vi "test elicitation.vi"(8 "error in (no error)":errorcluster) -> (0 "error out":errorcluster, 3 "body":string)   [LabVIEW 2020, in "MCP Server tests.lvlib"]
doc: "Elicitation with the multi round-trip pattern of MCP 2026-07-28. fake_tool_confirm calls Confirm With User.vi with the key confirm_action. A modern call from a client with the elicitation capability gets resultType input_required with inputRequests.confirm_action (elicitation/create, form mode); the retry with inputResponses accept runs the confirmed path, decline the declined path. Without the capability, and in the legacy era, the tool takes its not supported path. The requests are sent with the LabVIEW HTTP Client directly."
uses:
  MCP Server tests.lvlib
  <vilib>/JDP Science/JSONtext/Next JSON Value.vi
  <vilib>/JDP Science/JSONtext/String Subset.vi
  <vilib>/JDP Science/JSONtext/Parsing/Advance past next JSON Value (inlined COPY).vi
  <vilib>/JDP Science/JSONtext/Parsing/Advance past whitespace.vi
  <vilib>/JDP Science/JSONtext/Parsing/Advance past String.vi
  <vilib>/JDP Science/JSONtext/Parsing/Advance past Number.vi
  <vilib>/JDP Science/JSONtext/Parsing/Advance past Line Ending.vi
  <vilib>/JDP Science/JSONtext/Parsing/Parse Full Path or Item Name.vi
  <vilib>/JDP Science/JSONtext/Parsing/Advance past Array.vi
  <vilib>/JDP Science/JSONtext/Parsing/Advance past Object.vi
  <vilib>/JDP Science/JSONtext/support/Error Cluster From Code.vi
  <vilib>/JDP Science/JSONtext/Offset/Find Item Locations by Path.vi
  <vilib>/addons/_JKI Toolkits/Caraya/classes/Test/Test.lvclass
  <vilib>/JDP Science/JSONtext/JSONtext.lvlib
  <vilib>/addons/_JKI Toolkits/Caraya/classes/Assert/Assert.lvclass
panel:
  out "lookup error":errorcluster
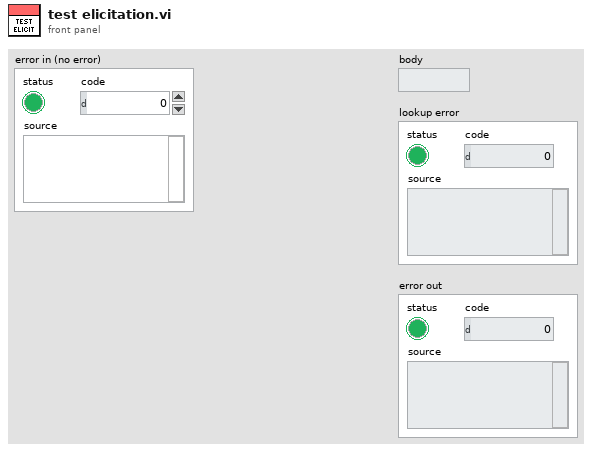
[diagram p1: front panel]
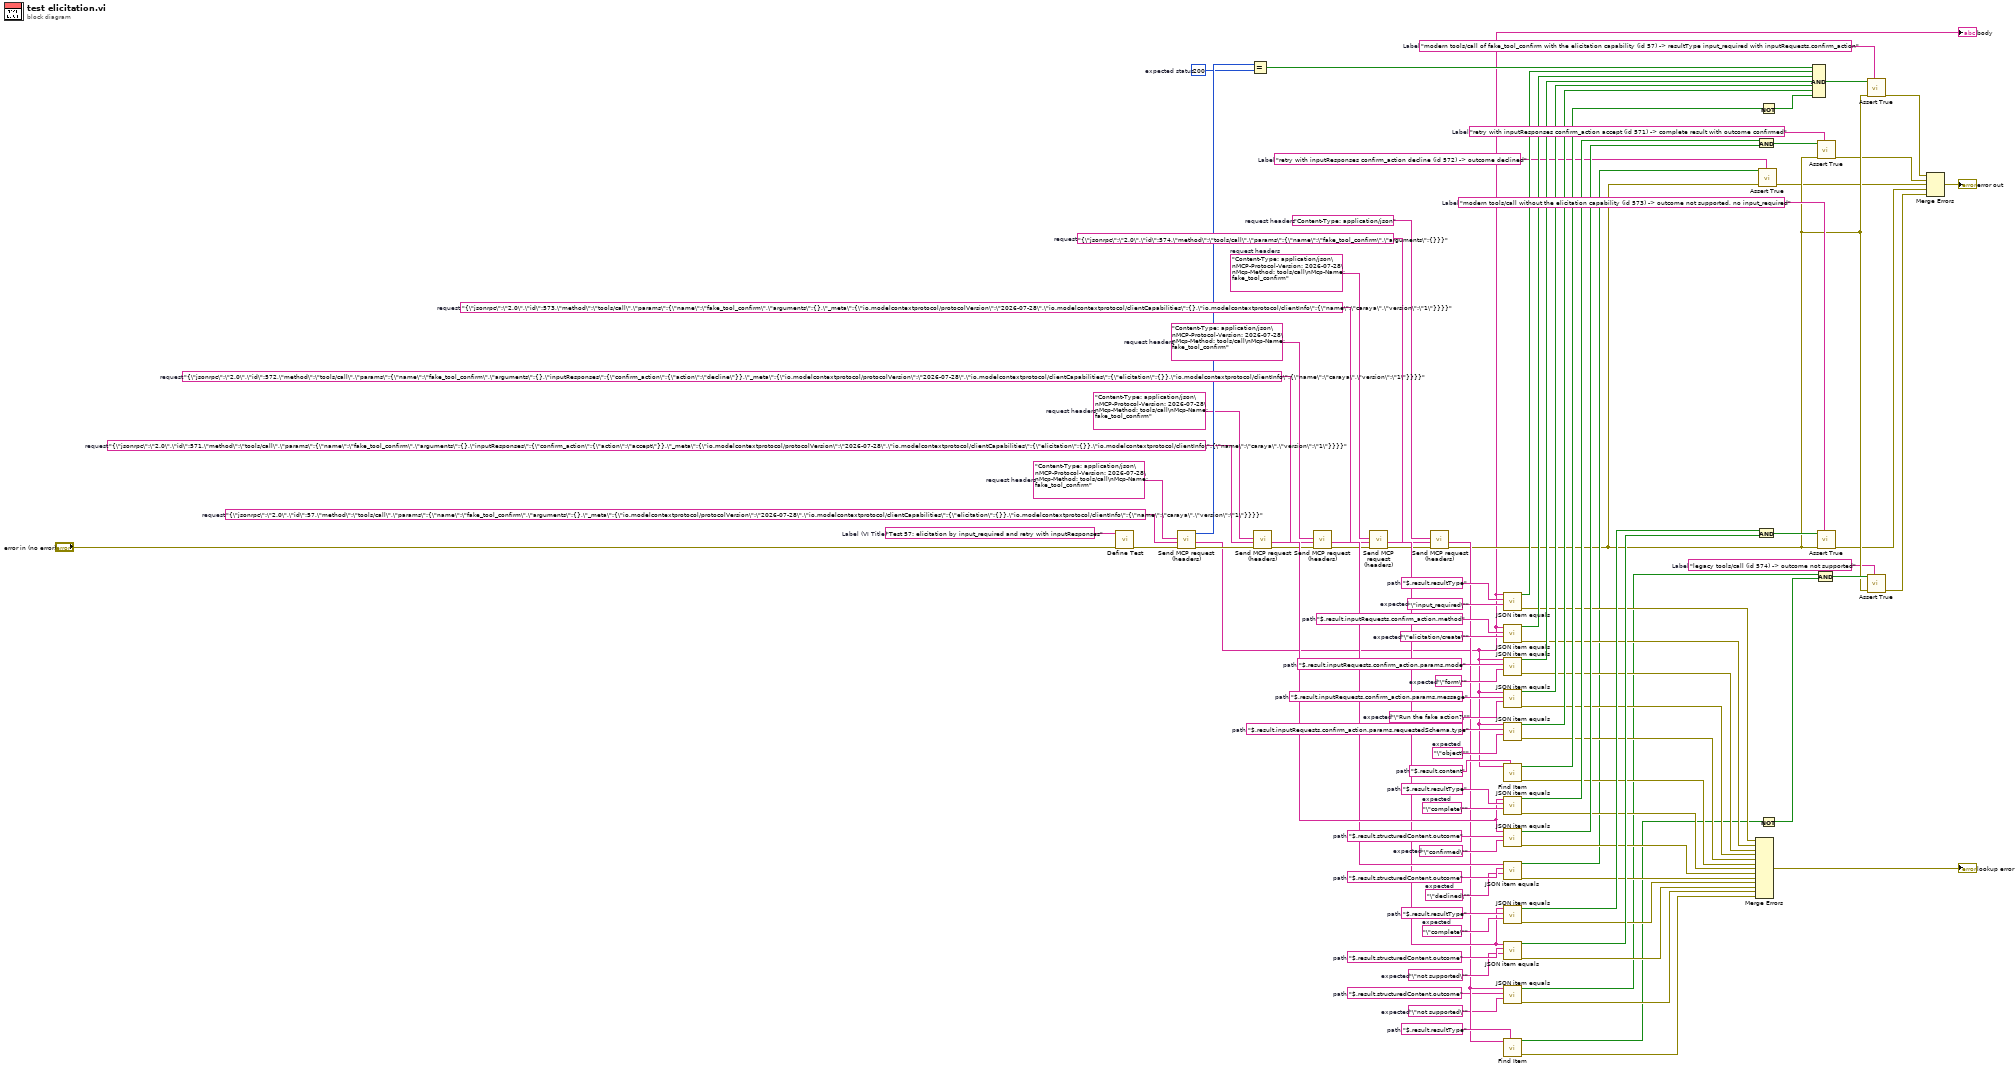
[diagram p0: block diagram]
diagram:
  w42 = "Content-Type: application/json"  # request headers
  w52 = "Content-Type: application/json\nMCP-Protocol-Version: 2026-07-28\nMcp-Method: tools/call\nMcp-Name: fake_tool_confirm"  # request headers
  w58 = "Content-Type: application/json\nMCP-Protocol-Version: 2026-07-28\nMcp-Method: tools/call\nMcp-Name: fake_tool_confirm"  # request headers
  w68 = "Content-Type: application/json\nMCP-Protocol-Version: 2026-07-28\nMcp-Method: tools/call\nMcp-Name: fake_tool_confirm"  # request headers
  w92 = "Content-Type: application/json\nMCP-Protocol-Version: 2026-07-28\nMcp-Method: tools/call\nMcp-Name: fake_tool_confirm"  # request headers
  w9 = "legacy tools/call (id 574) -> outcome not supported"  # Label
  w14 = "modern tools/call without the elicitation capability (id 573) -> outcome not supported, no input_required"  # Label
  w16 = "retry with inputResponses confirm_action decline (id 572) -> outcome declined"  # Label
  w18 = "retry with inputResponses confirm_action accept (id 571) -> complete result with outcome confirmed"  # Label
  w20 = "modern tools/call of fake_tool_confirm with the elicitation capability (id 57) -> resultType input_required with inputRequests.confirm_action"  # Label
  w39 = "$.result.resultType"  # path
  w36 = "\"not supported\""  # expected
  w37 = "$.result.structuredContent.outcome"  # path
  w45 = "\"not supported\""  # expected
  w46 = "$.result.structuredContent.outcome"  # path
  w48 = "\"complete\""  # expected
  w49 = "$.result.resultType"  # path
  w53 = "\"declined\""  # expected
  w54 = "$.result.structuredContent.outcome"  # path
  w61 = "\"confirmed\""  # expected
  w62 = "$.result.structuredContent.outcome"  # path
  w64 = "\"complete\""  # expected
  w65 = "$.result.resultType"  # path
  w89 = "$.result.content"  # path
  w79 = "\"object\""  # expected
  w80 = "$.result.inputRequests.confirm_action.params.requestedSchema.type"  # path
  w81 = "\"Run the fake action?\""  # expected
  w82 = "$.result.inputRequests.confirm_action.params.message"  # path
  w83 = "\"form\""  # expected
  w84 = "$.result.inputRequests.confirm_action.params.mode"  # path
  w85 = "\"elicitation/create\""  # expected
  w86 = "$.result.inputRequests.confirm_action.method"  # path
  w87 = "\"input_required\""  # expected
  w88 = "$.result.resultType"  # path
  w76 = 200  # expected status
  w41 = "{\"jsonrpc\":\"2.0\",\"id\":574,\"method\":\"tools/call\",\"params\":{\"name\":\"fake_tool_confirm\",\"arguments\":{}}}"  # request
  w51 = "{\"jsonrpc\":\"2.0\",\"id\":573,\"method\":\"tools/call\",\"params\":{\"name\":\"fake_tool_confirm\",\"arguments\":{},\"_meta\":{\"io.modelcontextprotocol/protocolVersion\":\"2026-07-28\",\"io.modelcontextprotocol/clientCapabilities\":{},\"io.modelcontextprotocol/clientInfo\":{\"name\":\"caraya\",\"version\":\"1\"}}}}"  # request
  w57 = "{\"jsonrpc\":\"2.0\",\"id\":572,\"method\":\"tools/call\",\"params\":{\"name\":\"fake_tool_confirm\",\"arguments\":{},\"inputResponses\":{\"confirm_action\":{\"action\":\"decline\"}},\"_meta\":{\"io.modelcontextprotocol/protocolVersion\":\"2026-07-28\",\"io.modelcontextprotocol/clientCapabilities\":{\"elicitation\":{}},\"io.modelcontextprotocol/clientInfo\":{\"name\":\"caraya\",\"version\":\"1\"}}}}"  # request
  w67 = "{\"jsonrpc\":\"2.0\",\"id\":571,\"method\":\"tools/call\",\"params\":{\"name\":\"fake_tool_confirm\",\"arguments\":{},\"inputResponses\":{\"confirm_action\":{\"action\":\"accept\"}},\"_meta\":{\"io.modelcontextprotocol/protocolVersion\":\"2026-07-28\",\"io.modelcontextprotocol/clientCapabilities\":{\"elicitation\":{}},\"io.modelcontextprotocol/clientInfo\":{\"name\":\"caraya\",\"version\":\"1\"}}}}"  # request
  w91 = "{\"jsonrpc\":\"2.0\",\"id\":57,\"method\":\"tools/call\",\"params\":{\"name\":\"fake_tool_confirm\",\"arguments\":{},\"_meta\":{\"io.modelcontextprotocol/protocolVersion\":\"2026-07-28\",\"io.modelcontextprotocol/clientCapabilities\":{\"elicitation\":{}},\"io.modelcontextprotocol/clientInfo\":{\"name\":\"caraya\",\"version\":\"1\"}}}}"  # request
  w94 = "Test 57: elicitation by input_required and retry with inputResponses"  # Label (VI Title)
  n1 = call <vilib>:"Define Test.vi"("error in (no error)"="error in (no error)", "Label (VI Title)"=w94) -> ("error out"=w90:errorcluster)  [unwired: 8 in, 1 out]
  n2 = call "Send MCP request (headers).vi"("error in (no error)"=w90, "request"=w91, "request headers"=w92) -> ("error out"=w66:errorcluster, "response"=w3:string, "status code"=w77:i32)  [unwired: 5 in, 1 out]
  "body" <- w3
  n3 = Equal?(x=w77, y=w76) -> (x = y?=w75:bool)
  n4 = call "Send MCP request (headers).vi"("error in (no error)"=w66, "request"=w67, "request headers"=w68) -> ("error out"=w56:errorcluster, "response"=w63:string)  [unwired: 5 in, 2 out]
  n5 = call "Send MCP request (headers).vi"("error in (no error)"=w56, "request"=w57, "request headers"=w58) -> ("error out"=w50:errorcluster, "response"=w55:string)  [unwired: 5 in, 2 out]
  n6 = call "Send MCP request (headers).vi"("error in (no error)"=w50, "request"=w51, "request headers"=w52) -> ("error out"=w40:errorcluster, "response"=w47:string)  [unwired: 5 in, 2 out]
  n7 = call "Send MCP request (headers).vi"("error in (no error)"=w40, "request"=w41, "request headers"=w42) -> ("error out"=w10:errorcluster, "response"=w38:string)  [unwired: 5 in, 2 out]
  n8 = call "JSON item equals.vi"("expected"=w87, "path"=w88, "JSON"=w3) -> ("error out"=w35:errorcluster, "equal?"=w74:bool)  [unwired: 6 in, 1 out]
  n9 = call "JSON item equals.vi"("expected"=w85, "path"=w86, "JSON"=w3) -> ("error out"=w34:errorcluster, "equal?"=w73:bool)  [unwired: 6 in, 1 out]
  n10 = call "JSON item equals.vi"("expected"=w83, "path"=w84, "JSON"=w3) -> ("error out"=w33:errorcluster, "equal?"=w72:bool)  [unwired: 6 in, 1 out]
  n11 = call "JSON item equals.vi"("expected"=w81, "path"=w82, "JSON"=w3) -> ("error out"=w32:errorcluster, "equal?"=w71:bool)  [unwired: 6 in, 1 out]
  n12 = call "JSON item equals.vi"("expected"=w79, "path"=w80, "JSON"=w3) -> ("error out"=w31:errorcluster, "equal?"=w70:bool)  [unwired: 6 in, 1 out]
  n13 = call <vilib>:"Find Item.vi"("$Path or Item Name"=w89, "JSON"=w3) -> ("error out"=w30:errorcluster, "Found"=w78:bool)  [unwired: 6 in, 2 out]
  n14 = call "JSON item equals.vi"("expected"=w64, "path"=w65, "JSON"=w63) -> ("error out"=w29:errorcluster, "equal?"=w60:bool)  [unwired: 6 in, 1 out]
  n15 = call "JSON item equals.vi"("expected"=w61, "path"=w62, "JSON"=w63) -> ("error out"=w28:errorcluster, "equal?"=w59:bool)  [unwired: 6 in, 1 out]
  n16 = call "JSON item equals.vi"("expected"=w53, "path"=w54, "JSON"=w55) -> ("error out"=w27:errorcluster, "equal?"=w17:bool)  [unwired: 6 in, 1 out]
  n17 = call "JSON item equals.vi"("expected"=w48, "path"=w49, "JSON"=w47) -> ("error out"=w26:errorcluster, "equal?"=w44:bool)  [unwired: 6 in, 1 out]
  n18 = call "JSON item equals.vi"("expected"=w45, "path"=w46, "JSON"=w47) -> ("error out"=w25:errorcluster, "equal?"=w43:bool)  [unwired: 6 in, 1 out]
  n19 = call "JSON item equals.vi"("expected"=w36, "path"=w37, "JSON"=w38) -> ("error out"=w24:errorcluster, "equal?"=w13:bool)  [unwired: 6 in, 1 out]
  n20 = call <vilib>:"Find Item.vi"("$Path or Item Name"=w39, "JSON"=w38) -> ("error out"=w23:errorcluster, "Found"=w22:bool)  [unwired: 6 in, 2 out]
  n21 = Merge Errors(w35, w34, w33, w32, w31, w30, w29, w28, w27, w26, w25, w24, w23) -> (→"lookup error":errorcluster)
  n22 = call <vilib>:"Assert True.vi"("Label"=w16, "error in (no error)"=w10, "True?"=w17) -> ("error out"=w6:errorcluster)  [unwired: 7 in, 1 out]
  n23 = Not(x=w78) -> (.not. x?=w69:bool)
  n24 = Compound Arithmetic op=AND(w60, w59) -> (w19:bool)
  n25 = Compound Arithmetic op=AND(w44, w43) -> (w15:bool)
  n26 = Not(x=w22) -> (.not. x?=w12:bool)
  n27 = Compound Arithmetic op=AND(w75, w74, w73, w72, w71, w70, w69) -> (w21:bool)
  n28 = call <vilib>:"Assert True.vi"("Label"=w18, "error in (no error)"=w10, "True?"=w19) -> ("error out"=w7:errorcluster)  [unwired: 7 in, 1 out]
  n29 = call <vilib>:"Assert True.vi"("Label"=w14, "error in (no error)"=w10, "True?"=w15) -> ("error out"=w5:errorcluster)  [unwired: 7 in, 1 out]
  n30 = Compound Arithmetic op=AND(w13, w12) -> (w11:bool)
  n31 = call <vilib>:"Assert True.vi"("Label"=w20, "error in (no error)"=w10, "True?"=w21) -> ("error out"=w8:errorcluster)  [unwired: 7 in, 1 out]
  n32 = call <vilib>:"Assert True.vi"("Label"=w9, "error in (no error)"=w10, "True?"=w11) -> ("error out"=w4:errorcluster)  [unwired: 7 in, 1 out]
  n33 = Merge Errors(w8, w7, w6, w5, w4) -> (→"error out":errorcluster)
